vi "VIH HelpGen - Palette - Get All Sub-Menus.vi"(8 "error in":errorcluster, 10 "Include master menu (T)":bool=TRUE, 11 "Palette Path":path) -> (0 "error out":errorcluster, 2 "Palette Paths":path[](array[path]))   [LabVIEW 2014]
doc: "::: VI Helpeks :::\nCopyright (c) 2000-2026 Konstantin Shifershteyn. All rights reserved."
panel:
  # "VI Helpeks\nCopyright (c) 2012-2026 Konstantin Shifershteyn"
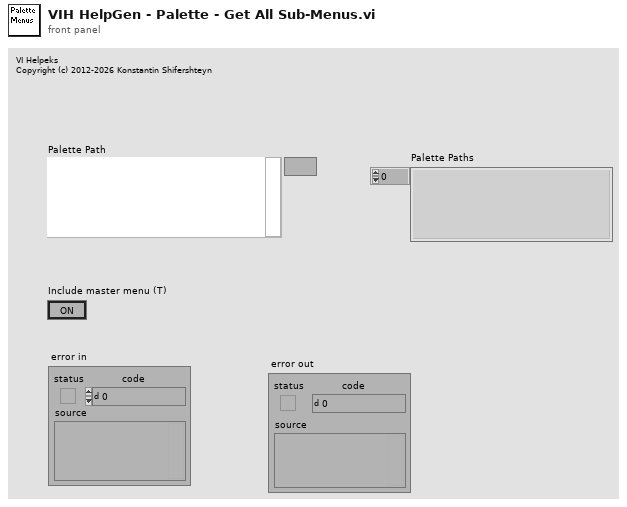
[diagram p1: front panel]
types:
  T1 = typedef "VIH HelpGen Typedef - Palette - Item Info Cluster.ctl" = cluster{"Item Type":T2, "Item Name":string, "Item File":path, "Parent palette":path, "Not found":bool}
  T2 = typedef "VIH HelpGen Typedef - Palette - Item Type Enum.ctl" = enum32{"<Invalid>", "<unknown>", "VI", "Menu", "LV Func", "Express VI", "Poly VI", "CTL", "HTML"}
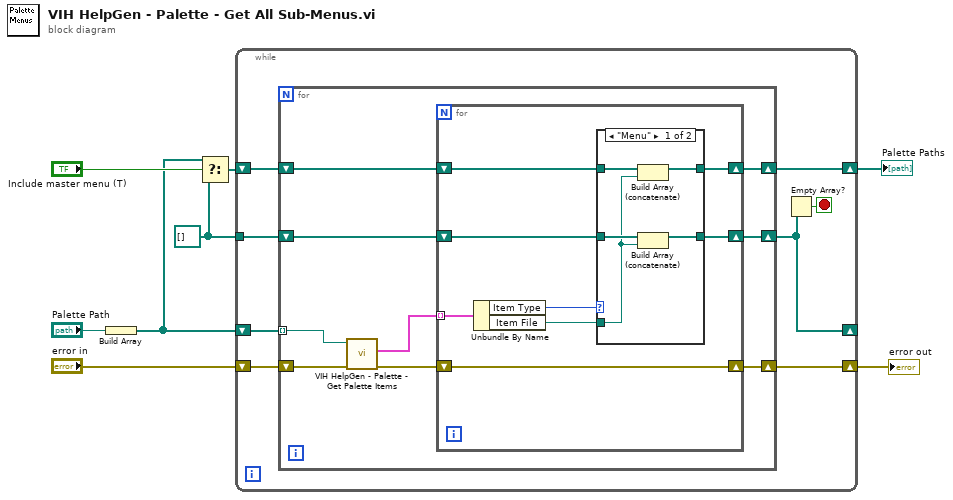
[diagram p0: block diagram]
diagram:
  w1 = path[] []
  n1 = Build Array("Palette Path") -> (w3:path[])
  n2 = Select(t=w3, s="Include master menu (T)", f=w1) -> (s? t:f=w2:path[])
  n3 = while {
    shift-right: [w13] -> _
    shift-left: w3 -> [w16]
    shift-right: [w14] -> w8
    shift-left: w2 -> [w15]
    shift-right: [w10] -> w7
    shift-left: "error in" -> [w11]
    tunnel: w1 -> [w9]
    stop <- w12 stop-if-true
    n4 = for {
      tunnel: w16 -> [w19] mode=indexing
      shift-right: [w21] -> w14
      shift-left: w15 -> [w22]
      shift-right: [w24] -> w13
      shift-left: w9 -> [w25]
      shift-right: [w23] -> w10
      shift-left: w11 -> [w20]
      n5 = call "VIH HelpGen - Palette - Get Palette Items.vi"("error in"=w20, "Palette Path"=w19) -> ("error out"=w17:errorcluster, "Items Array"=w18:T1[])  [unwired: 7 in, 1 out]
      n6 = for {
        tunnel: w18 -> [w33] mode=indexing
        shift-right: [w30] -> w24
        shift-left: w25 -> [w31]
        shift-right: [w29] -> w23
        shift-left: w17 -> [w29]
        shift-right: [w26] -> w21
        shift-left: w22 -> [w27]
        n7 = Unbundle By Name(w33) -> ("Item Type"=w32:T2, "Item File"=w28:path)
        n8 = case shown="\"Menu\"" w32 {
          tunnel: w31 -> [w38 w40]
          tunnel: [w37 w40] -> w30
          tunnel: w28 -> [w35 _]
          tunnel: w27 -> [w36 w39]
          tunnel: [w34 w39] -> w26
          frame "Menu" {
            n9 = Build Array (concatenate)(w36, w35) -> (w34:path[])
            n10 = Build Array (concatenate)(w38, w35) -> (w37:path[])
          }
          frame Default {
          }
        }
      }
    }
    n11 = Empty Array?(array=w13) -> (empty?=w12:bool)
  }
  "Palette Paths" <- w8
  "error out" <- w7
